vi "Write Numeric Output.vi"(8 "error in (no error)":errorcluster, 9 "Register Values":u16[](array[numeric]), 10 "Numeric Output":T1, 11 "Modbus in":refnum<class "Modbus.lvclass">) -> (0 "error out":errorcluster, 3 "Modbus out":refnum<class "Modbus.lvclass">)   [LabVIEW 2026, in "Modbus.lvlib" / "Modbus.lvclass"]
uses:
  Modbus.lvclass
  Types/Numeric Data.ctl
  Types/Modbus Table.ctl
  Types/Numeric Size.ctl
  Types/Numeric Data Type.ctl
  Types/Numeric Location.ctl
  Modbus.lvclass/Modbus.ctl
  <vilib>/ni/Modbus Library/API/Master/Modbus Master.lvclass
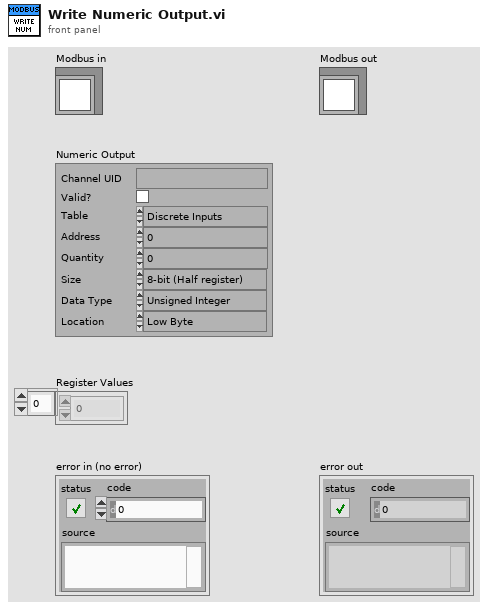
[diagram p1: front panel]
types:
  T1 = typedef "Modbus.lvlib/Modbus.lvclass/Numeric Data.ctl" = cluster{"Channel UID":string, "Valid?":bool, "Table":T2, "Address":i32, "Quantity":u16, "Size":T3, "Data Type":T4, "Location":T5}
  T2 = typedef "Modbus.lvlib/Modbus.lvclass/Modbus Table.ctl" = enum16{"Discrete Inputs", "Coils", "Input Registers", "Holding Registers"}
  T3 = typedef "Modbus.lvlib/Modbus.lvclass/Numeric Size.ctl" = enum16{"8-bit (Half register)", "16-bit (One register)", "32-bit (Two registers)", "64-bit (Four registers)"}
  T4 = typedef "Modbus.lvlib/Modbus.lvclass/Numeric Data Type.ctl" = enum16{"Unsigned Integer", "Signed Integer", "Floating Point"}
  T5 = typedef "Modbus.lvlib/Modbus.lvclass/Numeric Location.ctl" = enum16{"Low Byte", "High Byte"}
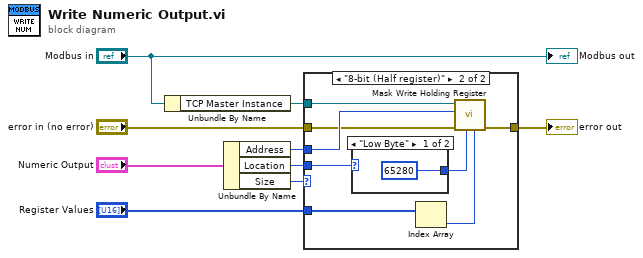
[diagram p0: block diagram]
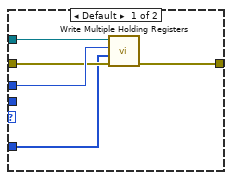
[diagram p2: hidden frame]
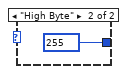
[diagram p3: hidden frame]
diagram:
  n1 = Unbundle By Name("Modbus in") -> ("TCP Master Instance"=w4:refnum<class "Modbus Master.lvclass">)
  n2 = Unbundle By Name("Numeric Output") -> ("Address"=w3:i32, "Location"=w2:T5, "Size"=w1:T3)
  n3 = case shown="\"8-bit (Half register)\"" w1 {
    tunnel: w4 -> [w14 w22]
    tunnel: w3 -> [w13 w21]
    tunnel: [w12 w20] -> w9
    tunnel: "error in (no error)" -> [w11 w19]
    tunnel: "Register Values" -> [w10 w18]
    tunnel: w2 -> [_ w16]
    frame Default {
      n4 = call-dynamic "Write Multiple Holding Registers.vi"("error in"=w11, "registers to write"=w10, "starting address"=w13, "Modbus master in"=w14) -> ("error out"=w12:errorcluster)  [unwired: 6 in, 1 out]
    }
    frame "8-bit (Half register)" {
      n5 = case shown="\"Low Byte\"" w16 {
        tunnel: [u16 65280 u16 255] -> w15
        frame "Low Byte" {
        }
        frame "High Byte" {
        }
      }
      n6 = Index Array(array=w18) -> (element=w17:u16)  [unwired: 1 in]
      n7 = call-dynamic "Mask Write Holding Register.vi"("OR Mask"=w17, "AND Mask"=w15, "error in"=w19, "address"=w21, "Modbus instance in"=w22) -> ("error out"=w20:errorcluster)  [unwired: 5 in, 1 out]
    }
  }
  "error out" <- w9
  "Modbus out" <- "Modbus in"
